vi "Fault Insertion UI.vi"() -> ()   [LabVIEW 2021]
uses:
  <vilib>/TSA/Omni-Bus/Fault-Injection Bus/Fault-Injection Bus.lvclass
  C:/Program Files (x86)/National Instruments/LabVIEW 2021/vi.lib/TSA/Omni-Bus/Omni-Bus/Bus Access/Bus_Access.lvclass
  <vilib>/TSA/Omni-Bus/Omni-Bus/Omni_Bus.lvclass
  <vilib>/TSA/Omni-Bus/Fault-Injection Bus/Support/Omni-Bus/Omni-Bus Inject DBL.vi
  <vilib>/TSA/Omni-Bus/Fault-Injection Bus/Support/Omni-Bus/Omni-Bus Inject Boolean.vi
  <vilib>/TSA/Omni-Bus/Fault-Injection Bus/Support/Value Type/DBL/Fault-Injection_DBL.lvclass
  C:/Program Files (x86)/National Instruments/LabVIEW 2021/vi.lib/TSA/Abstract Data Classes/Abs_Types/Type/Abs_Type.lvclass
  <vilib>/TSA/Omni-Bus/Fault-Injection Bus/Support/Value Type/Boolean/Fault-Injection_Boolean.lvclass
  <vilib>/TSA/Omni-Bus/Omni-Bus/Support/FindVar.vi
panel:
  in  "Fault-Injection Bus":refnum<class "Fault-Injection Bus.lvclass">
  in  "Enable Fault Heater State":bool
  in  "Fault Heater State":bool
  in  "Arm Fault Insertion":bool
  in  "Enable Fault Temp":bool
  in  "Fault Temp":dbl(slide) scale=20.0..80.0
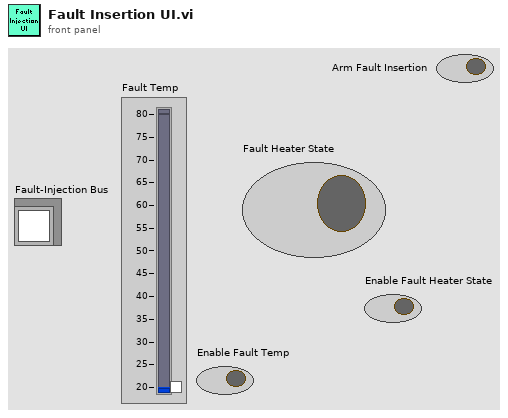
[diagram p1: front panel]
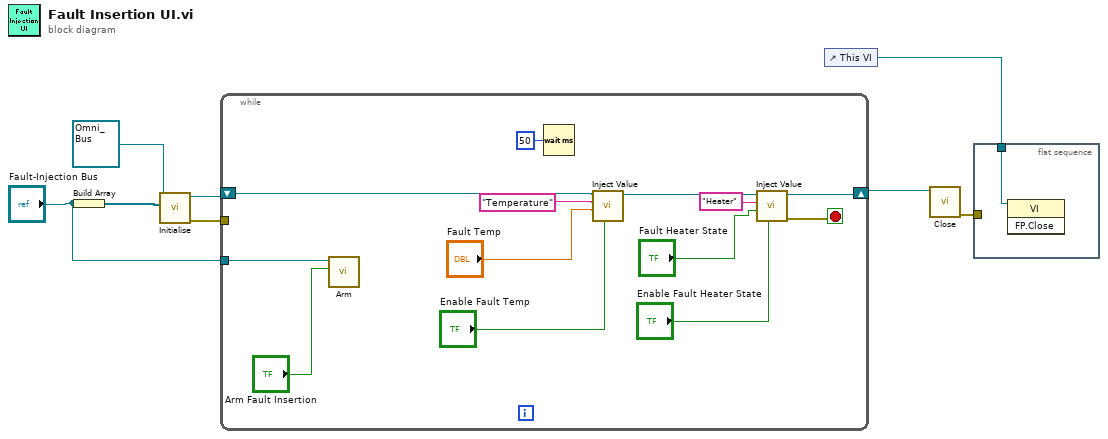
[diagram p0: block diagram]
diagram:
  n1 = Build Array("Fault-Injection Bus") -> (w2:refnum<class "Fault-Injection Bus.lvclass">[])
  n2 = call-dynamic "Initialise.vi"("Bus Access"=w2, "Var Bus in"=refnum<class "Omni_Bus.lvclass"> refnum) -> ("error out"=w5:errorcluster, "Var Bus out"=w7:refnum<class "Omni_Bus.lvclass">)  [unwired: 8 in]
  n3 = while {
    shift-right: [w14] -> w6
    shift-left: w7 -> [w19]
    tunnel: w5 -> [_]
    tunnel: "Fault-Injection Bus" -> [w10]
    stop <- w12 stop-if-true
    n4 = call <vilib>:"Arm.vi"("Arm"="Arm Fault Insertion", "Fault-Injection Bus in"=w10) -> ()  [unwired: 8 in, 2 out]
    n5 = Wait (ms)(milliseconds to wait=u32 50) -> ()  [unwired: 1 out]
    n6 = call-poly <vilib>:"Inject Value.vi"("Enable"="Enable Fault Temp", "Injected Value"="Fault Temp", "Tag"="Temperature", "Omni_Bus in"=w19) -> ("Omni_Bus out"=w16:refnum<class "Omni_Bus.lvclass">)  [unwired: 6 in, 1 out]
    n7 = call-poly <vilib>:"Inject Value.vi"("Enable"="Enable Fault Heater State", "Injected Value"="Fault Heater State", "Tag"="Heater", "Omni_Bus in"=w16) -> ("error out"=w12:errorcluster, "Omni_Bus out"=w14:refnum<class "Omni_Bus.lvclass">)  [unwired: 6 in]
  }
  n8 = control-ref of="This VI"() -> (w4:refnum<vi>)
  n9 = call-dynamic "Close.vi"("Data in"=w6) -> ("error out"=w3:errorcluster)  [unwired: 9 in, 1 out]
  n10 = flat-sequence {
    tunnel: w4 -> [w22]
    tunnel: w3 -> [_]
    frame #0 {
      n11 = invoke class="VI" method="FP.Close"(reference=w22) -> ()  [unwired: 2 in, 3 out]
    }
  }
